vi "Inline Temporary SubVIs.vi"(8 "error in (no error)":errorcluster, 11 "Responsive Mock Class Generator in":refnum<class "Mock Class Generator.lvclass">) -> (0 "error out":errorcluster, 3 "Responsive Mock Class Generator out":refnum<class "Mock Class Generator.lvclass">)   [LabVIEW 2020, in "Mock Class Generator.lvclass"]
uses:
  Mock Class Generator.lvclass
  Mock Class Generator.lvclass/Mock Class Generator.ctl
  Append Control Value.vi
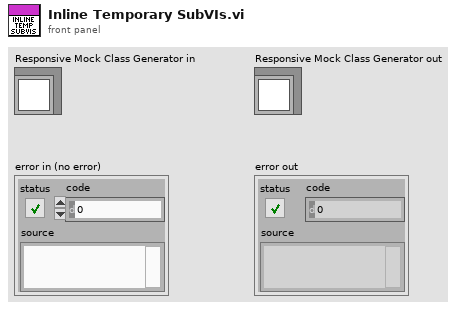
[diagram p1: front panel]
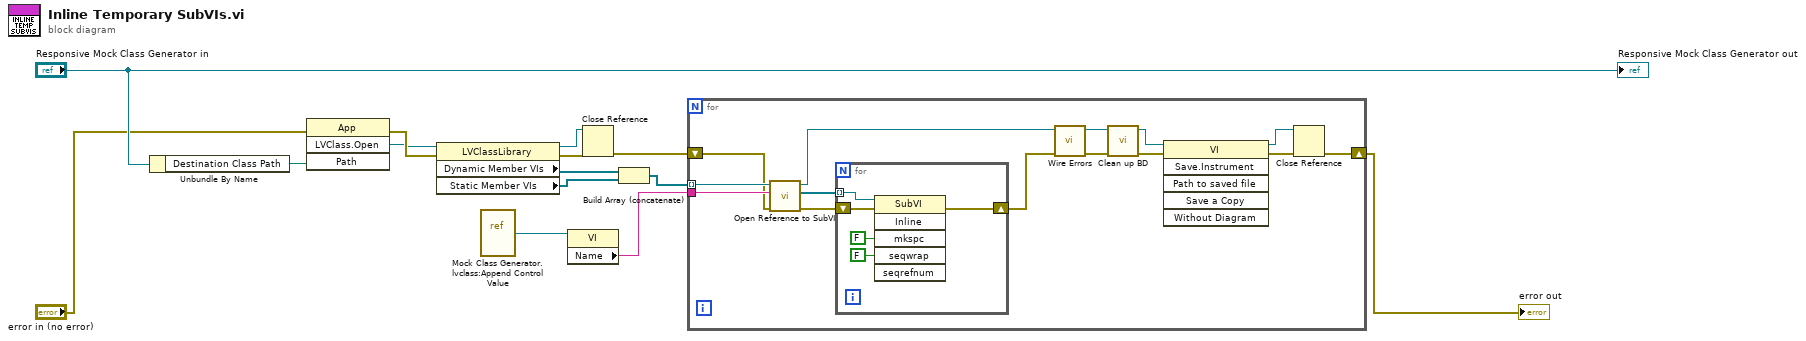
[diagram p0: block diagram]
diagram:
  n1 = Unbundle By Name("Responsive Mock Class Generator in") -> ("Destination Class Path"=w14:path)
  n2 = invoke class="App" method="LVClass.Open"(error in="error in (no error)", "Path"=w14) -> (error out=w13:errorcluster, "LVClass.Open"=w10:refnum<vi>)  [unwired: 2 in, 2 out]
  n3 = property class="LVClassLibrary"(reference=w10, error in=w13) -> (reference out=w11:refnum<vi>, error out=w12:errorcluster, "Dynamic Member VIs"=w7:refnum<vi>[], "Static Member VIs"=w6:refnum<vi>[])
  n4 = vi-ref "Mock Class Generator.lvclass:Append Control Value.vi"() -> (w5:refnum<vi>)
  n5 = property class="VI"(reference=w5) -> ("Name"=w3:string)  [unwired: 1 in, 2 out]
  n6 = Close Reference(reference=w11, error in (no error)=w12) -> (error out=w2:errorcluster)
  n7 = Build Array (concatenate)(w7, w6) -> (w4:refnum<vi>[])
  n8 = for {
    tunnel: w4 -> [w28] mode=indexing
    tunnel: w3 -> [w27]
    shift-right: [w22] -> w1
    shift-left: w2 -> [w26]
    n9 = call "Open Reference to SubVI.vi"("error in (no error)"=w26, "SubVI Name"=w27, "VI in"=w28) -> ("error out"=w25:errorcluster, "SubVIs"=w24:refnum<vi>[], "VI out"=w18:refnum<vi>)  [unwired: 6 in]
    n10 = for {
      shift-right: [w32] -> w16
      shift-left: w25 -> [w33]
      tunnel: w24 -> [w31] mode=indexing
      n11 = invoke class="SubVI" method="Inline"(reference=w31, error in=w33, "mkspc"=FALSE ("Make Space in Block Diagram"), "seqwrap"=FALSE ("Wrap in Sequence")) -> (error out=w32:errorcluster)  [unwired: 2 in, 5 out]
    }
    n12 = call "Wire Errors.vi"("error in (no error)"=w16, "VI in"=w18) -> ("error out"=w15:errorcluster, "VI out"=w17:refnum<vi>)  [unwired: 8 in]
    n13 = call "Clean up BD.vi"("error in (no error)"=w15, "VI in"=w17) -> ("error out"=w23:errorcluster, "VI out"=w20:refnum<vi>)  [unwired: 8 in]
    n14 = invoke class="VI" method="Save.Instrument"(reference=w20, error in=w23) -> (reference out=w19:refnum<vi>, error out=w21:errorcluster)  [unwired: 4 in, 4 out]
    n15 = Close Reference(reference=w19, error in (no error)=w21) -> (error out=w22:errorcluster)
  }
  "error out" <- w1
  "Responsive Mock Class Generator out" <- "Responsive Mock Class Generator in"
